vi "check should fail.vi"() -> ()   [LabVIEW 2016]
uses:
  Source/JSON Value/JSON Value.lvclass
panel:
  out "Array":T1(array[cluster])
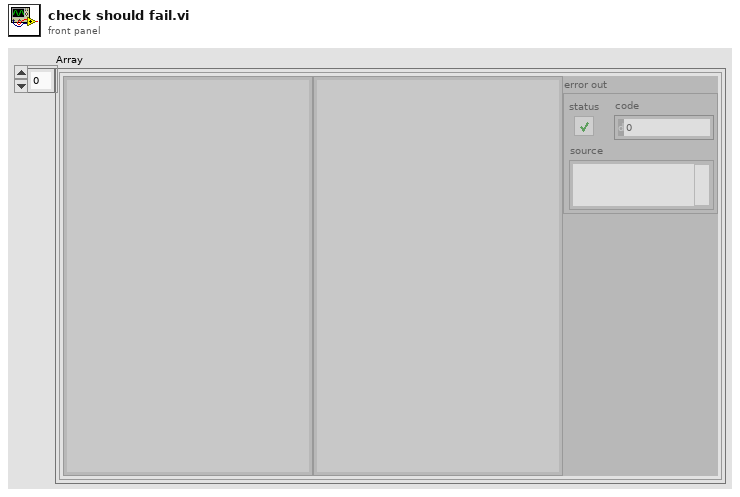
[diagram p1: front panel]
types:
  T1 = cluster{"String":string, string, "error out":errorcluster}[]
  T2 = cluster{"String":string, string, "error out":errorcluster}
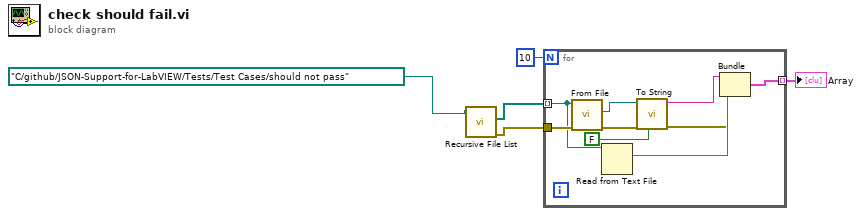
[diagram p0: block diagram]
diagram:
  n1 = call <vilib>:"Recursive File List.vi"("Folder Path"=path "C:/github/JSON-Support-for-LabVIEW/Tests/Test Cases/should not pass" ("Path")) -> ("error out"=w4:errorcluster, "All Files in Dir"=w2:path[])  [unwired: 6 in, 3 out]
  n2 = for {
    N: 10 -> [_]
    tunnel: w2 -> [w11] mode=indexing
    tunnel: w4 -> [w13]
    tunnel: [w8] -> w3 mode=indexing
    n3 = call "From File.vi"("error in"=w13, "file path"=w11) -> ("error out"=w12:errorcluster, "JSON Value out"=w14:refnum<class "JSON Value.lvclass">)  [unwired: 8 in]
    n4 = Read from Text File(file (use dialog)=w11) -> (text=w9:string)  [unwired: 3 in, 3 out]
    n5 = call "To String.vi"("pretty print? (T)"=FALSE, "error in (no error)"=w12, "JSON Value in"=w14) -> ("error out"=w7:errorcluster, "String"=w10:string)  [unwired: 7 in]
    n6 = Bundle("String"=w10, w9, "error out"=w7) -> (w8:T2)  [unwired: 1 in]
  }
  "Array" <- w3
